vi "Replace In Descriptions.vi"() -> ()   [LabVIEW 2020]
doc: "Dev helper: replaces text in the VI description of every VI listed in the items file (one path per line) and saves the VIs it changed. The pairs file holds one replacement per line, the text to find and its replacement separated by a tab; every occurrence is replaced, pairs applied in order. Run it in LabVIEW 2020 over Remote Run.vi so the VIs stay saved for 20.0. Returns per item whether the description changed and the error code."
panel:
  out "error out":errorcluster
  out "codes":i32[](array[numeric])
  out "changed":bool[](array[boolean])
  in  "pairs file":path
  in  "items file":path
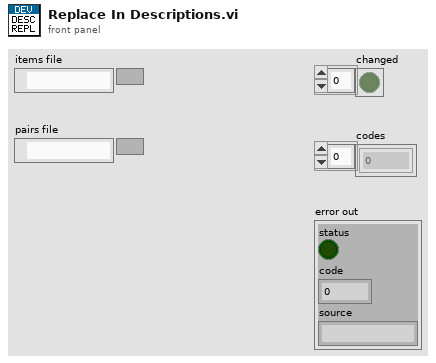
[diagram p1: front panel]
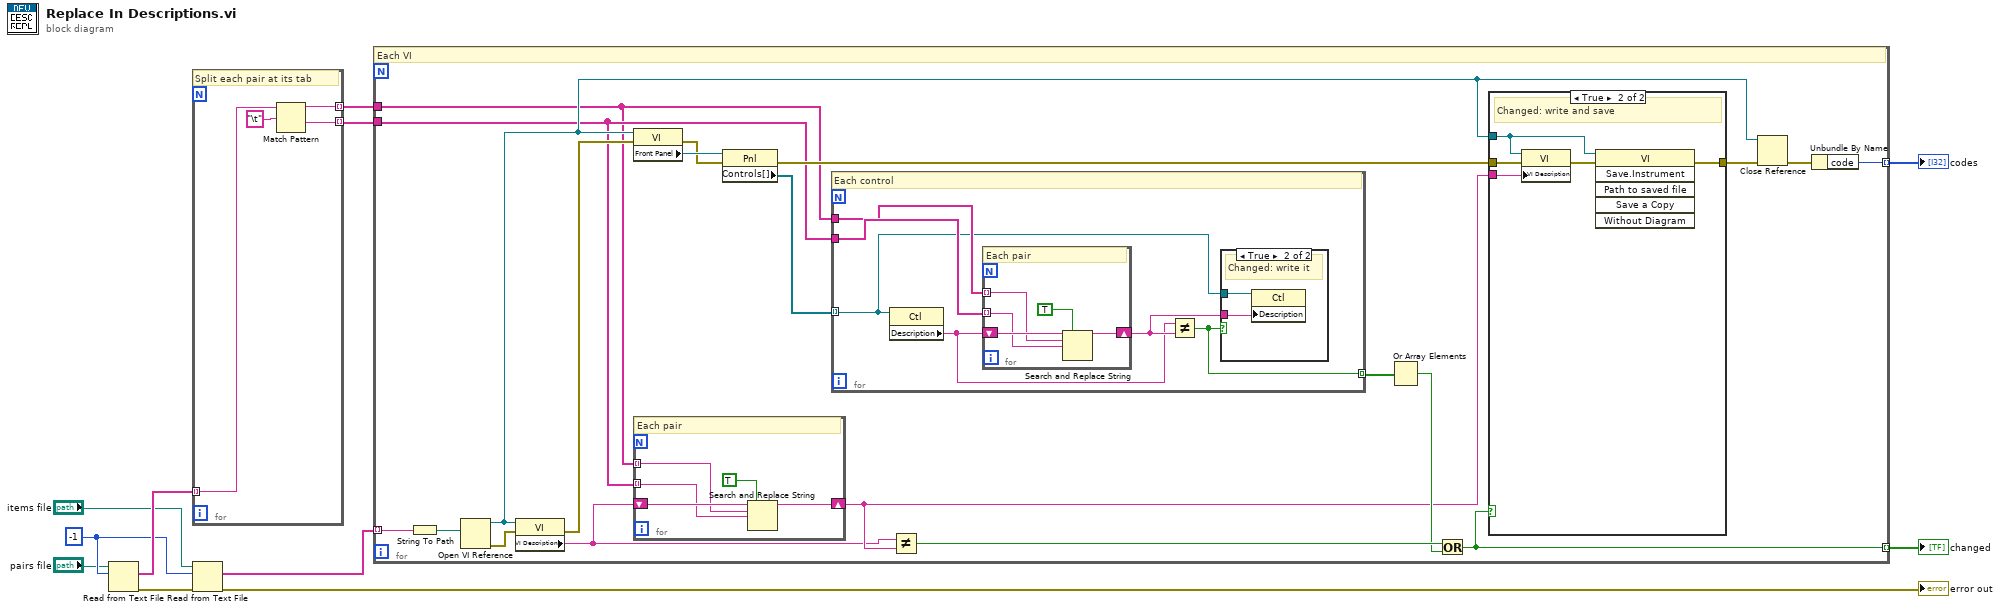
[diagram p0: block diagram]
diagram:
  w3 = -1
  n1 = Read from Text File(file (use dialog)="pairs file", count=w3) -> (text=w4:string[], error out=w5:errorcluster)  [unwired: 2 in, 2 out]
  n2 = for {
    tunnel: w4 -> [w12] mode=indexing
    tunnel: [w14] -> w6 mode=indexing
    tunnel: [w15] -> w7 mode=indexing
    # "Split each pair at its tab"
    n3 = Match Pattern(string=w12, regular expression="\t") -> (before substring=w14:string, after substring=w15:string)  [unwired: 1 in, 2 out]
  }
  n4 = Read from Text File(file (use dialog)="items file", count=w3, error in=w5) -> (text=w8:string[], error out=→"error out":errorcluster)  [unwired: 1 in, 2 out]
  n5 = for {
    tunnel: w8 -> [w16] mode=indexing
    tunnel: w6 -> [w17]
    tunnel: w7 -> [w18]
    tunnel: [w35] -> w10 mode=indexing
    tunnel: [w32] -> w11 mode=indexing
    # "Each VI"
    n6 = String To Path(string=w16) -> (path=w19:path)
    n7 = Open VI Reference(vi path=w19) -> (vi reference=w20:refnum<vi>, error out=w21:errorcluster)  [unwired: 5 in]
    n8 = property class="VI"(reference=w20, error in=w21) -> (error out=w22:errorcluster, "VI Description"=w23:string)  [unwired: 1 out]
    n9 = property class="VI"(reference=w20, error in=w22) -> (error out=w25:errorcluster, "Front Panel"=w26:refnum<vi>)  [unwired: 1 out]
    n10 = for {
      tunnel: w17 -> [w55] mode=indexing
      tunnel: w18 -> [w56] mode=indexing
      shift-right: [w58] -> w24
      shift-left: w23 -> [w57]
      # "Each pair"
      n11 = Search and Replace String(replace all?=TRUE, input string=w57, search string=w55, replace string=w56) -> (result string=w58:string)  [unwired: 4 in, 3 out]
    }
    n12 = property class="Pnl"(reference=w26, error in=w25) -> (error out=w27:errorcluster, "Controls[]"=w28:refnum<vi>[])  [unwired: 1 out]
    n13 = for {
      tunnel: w17 -> [w43]
      tunnel: w18 -> [w44]
      tunnel: w28 -> [w42] mode=indexing
      tunnel: [w47] -> w29 mode=indexing
      # "Each control"
      n14 = property class="Ctl"(reference=w42) -> ("Description"=w45:string)  [unwired: 1 in, 2 out]
      n15 = for {
        tunnel: w43 -> [w50] mode=indexing
        tunnel: w44 -> [w51] mode=indexing
        shift-right: [w53] -> w46
        shift-left: w45 -> [w52]
        # "Each pair"
        n16 = Search and Replace String(replace all?=TRUE, input string=w52, search string=w50, replace string=w51) -> (result string=w53:string)  [unwired: 4 in, 3 out]
      }
      n17 = Not Equal?(x=w45, y=w46) -> (x != y?=w47:bool)
      n18 = case shown="True" w47 {
        tunnel: w42 -> [_ w48]
        tunnel: w46 -> [_ w49]
        frame False {
          # "Unchanged"
        }
        frame True {
          # "Changed: write it"
          n19 = property class="Ctl"(reference=w48, "Description"=w49) -> ()  [unwired: 1 in, 2 out]
        }
      }
    }
    n20 = Not Equal?(x=w23, y=w24) -> (x != y?=w31:bool)
    n21 = Or Array Elements(Boolean array=w29) -> (logical OR=w30:bool)
    n22 = Or(x=w31, y=w30) -> (x .or. y?=w32:bool)
    n23 = case shown="True" w32 {
      tunnel: w20 -> [_ w37]
      tunnel: w24 -> [_ w39]
      tunnel: w27 -> [w36 w38]
      tunnel: [w36 w41] -> w33
      frame False {
        # "Unchanged"
      }
      frame True {
        # "Changed: write and save"
        n24 = property class="VI"(reference=w37, error in=w38, "VI Description"=w39) -> (error out=w40:errorcluster)  [unwired: 1 out]
        n25 = invoke class="VI" method="Save.Instrument"(reference=w37, error in=w40) -> (error out=w41:errorcluster)  [unwired: 4 in, 5 out]
      }
    }
    n26 = Close Reference(reference=w20, error in (no error)=w33) -> (error out=w34:errorcluster)
    n27 = Unbundle By Name(w34) -> ("code"=w35:i32)
  }
  "changed" <- w11
  "codes" <- w10
